vi "Scale By.vi"(0 "obj in":refnum<class "Can Scale.lvclass">, 1 "Factor":dbl=1.0) -> (2 "obj out":refnum<class "Can Scale.lvclass">)   [LabVIEW 2026, in "Can Scale.lvclass"]
doc: "Round14: the one method the interface Can Scale declares. obj in / obj out are path stand-ins that lvai_add_class_method retypes to the class; the diagram is a pass-through."
uses:
  Can Scale.lvclass
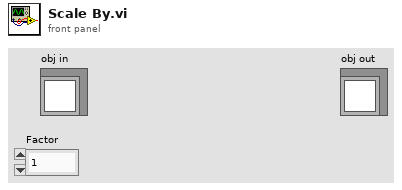
[diagram p1: front panel]
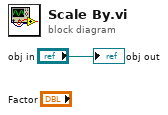
[diagram p0: block diagram]
diagram:
  "obj out" <- "obj in"
